vi "get target by alias.vi"(8 "error in":errorcluster, 10 "alias":string, 11 "system hierarchy":T1) -> (0 "error out":errorcluster, 3 "target hierarchy":T1)   [LabVIEW 2013, in "PL_Serialization Interface.lvlib"]
doc: "Searches a flattened instance data hierarhy for a specific target by the alias and returns the first target to match this alias, assuming that the current root element is the system level. If multiple targets share an alias, this selects the first. If the target is not found, error 538508 is returned."
uses:
  PL_Serialization Interface.lvlib
  <vilib>/NI/Configuration Framework/tree serializer/flat hierarchy.ctl
  <vilib>/NI/Configuration Framework/tree serializer/full hierarchy.ctl
  <vilib>/NI/Configuration Framework/tree serializer/hierarchy element.ctl
  <vilib>/NI/Configuration Framework/tree serializer/instance data.ctl
  <vilib>/NI/Configuration Framework/tree serializer/NISE_CEF_TreeSerializer.lvlib
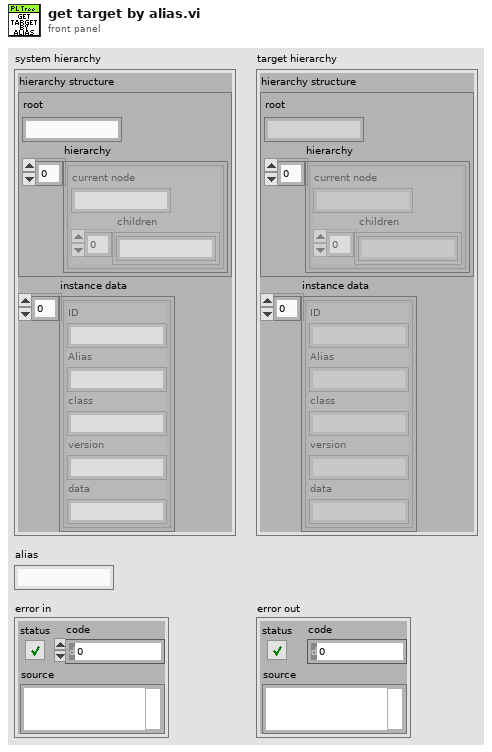
[diagram p1: front panel]
types:
  T1 = typedef "NISE_CEF_TreeSerializer.lvlib/flat hierarchy.ctl" = cluster{"hierarchy structure":T2, "instance data":T4[]}
  T2 = typedef "NISE_CEF_TreeSerializer.lvlib/full hierarchy.ctl" = cluster{"root":string, "hierarchy":T3[]}
  T3 = typedef "NISE_CEF_TreeSerializer.lvlib/hierarchy element.ctl" = cluster{"current node":string, "children":string[]}
  T4 = typedef "NISE_CEF_TreeSerializer.lvlib/instance data.ctl" = cluster{"ID":string, "Alias":string, "class":string, "version":string, "data":string}
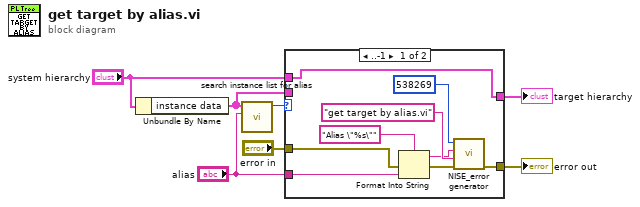
[diagram p0: block diagram]
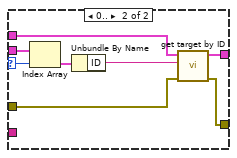
[diagram p2: hidden frame]
diagram:
  n1 = Unbundle By Name("system hierarchy") -> ("instance data"=w5:T4[])
  n2 = call <vilib>:"search instance list for alias.vi"("alias"="alias", "instance data"=w5) -> ("index"=w2:i32)  [unwired: 9 in]
  n3 = case shown="..-1" w2 {
    selector: w2 -> [_ w17]
    tunnel: "error in" -> [w15 w24]
    tunnel: [w14 w23] -> w6
    tunnel: w5 -> [_ w22]
    tunnel: "system hierarchy" -> [w16 w19]
    tunnel: [w16 w18] -> w3
    tunnel: "alias" -> [w10 _]
    frame ..-1 {
      n4 = Format Into String(format string="Alias \"%s\"", error in=w15, w10) -> (resulting string=w9:string, error out=w11:errorcluster)  [unwired: 1 in]
      n5 = call <vilib>:"NISE_error generator.vi"("error in"=w11, "source"="get target by alias.vi", "append error message"=w9, "error code (0)"=538269) -> ("error out"=w14:errorcluster)  [unwired: 5 in]
    }
    frame 0.. {
      n6 = Index Array(array=w22, index=w17) -> (element=w21:T4)
      n7 = Unbundle By Name(w21) -> ("ID"=w20:string)
      n8 = call "get target by ID.vi"("error in"=w24, "UID"=w20, "full system"=w19) -> ("error out"=w23:errorcluster, "target hierarchy"=w18:T1)  [unwired: 7 in]
    }
  }
  "error out" <- w6
  "target hierarchy" <- w3
